vi "Lockin.Low Pass Filter.vi"(8 "error in (no error)":errorcluster, 11 "DSP in":refnum<class "DSP.lvclass">) -> (0 "error out":errorcluster, 3 "DSP out":refnum<class "DSP.lvclass">)   [LabVIEW 2019, in "DSP.lvclass"]
uses:
  DSP.lvclass
  DSP.lvclass/DSP.ctl
panel:
  out "Waveforms out":T1
  out "Waveforms in":T1
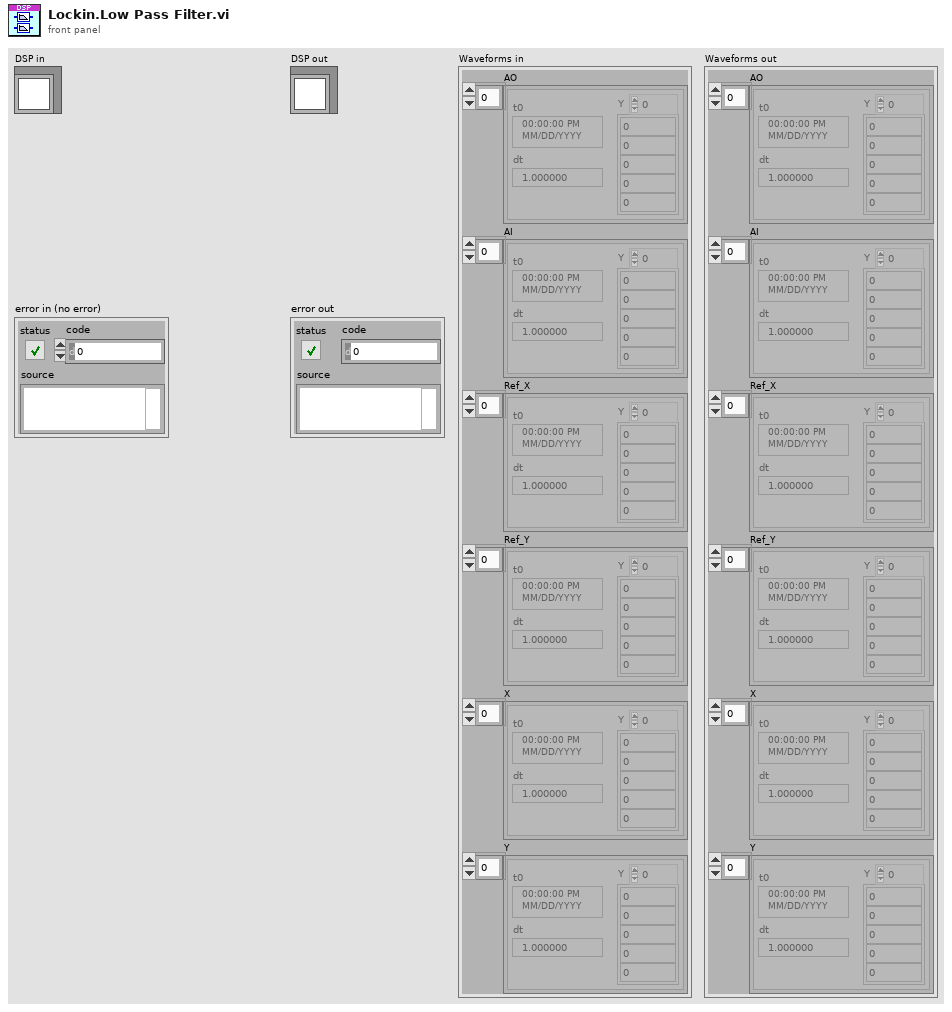
[diagram p1: front panel]
types:
  T1 = cluster{"AO":waveform(dbl)[], "AI":waveform(dbl)[], "Ref_X":waveform(dbl)[], "Ref_Y":waveform(dbl)[], "X":waveform(dbl)[], "Y":waveform(dbl)[]}
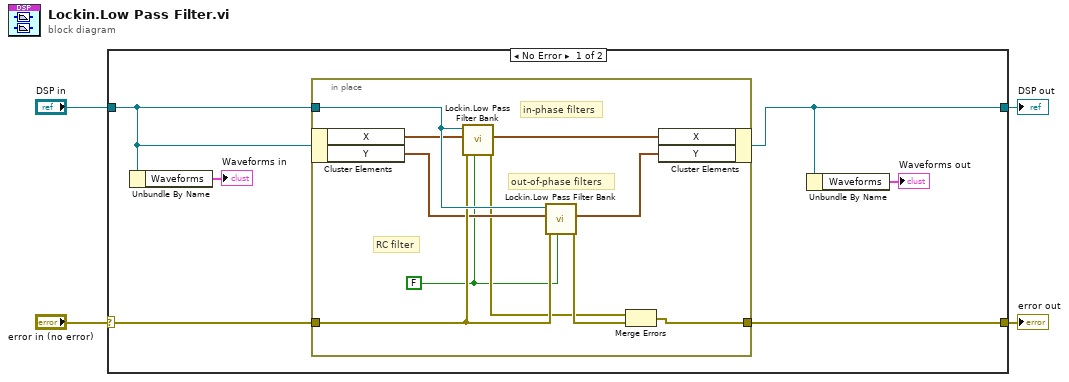
[diagram p0: block diagram]
diagram:
  n1 = case shown="No Error" "error in (no error)" {
    selector: "error in (no error)" -> [w9 w22]
    tunnel: [w10 w22] -> w4
    tunnel: [w5 w21] -> w3
    tunnel: "DSP in" -> [w7 w21]
    frame No Error {
      n2 = Unbundle By Name(w7) -> ("Waveforms"=→"Waveforms in":T1)
      n3 = in-place {
        in-place-border: [w20] -> w10
        in-place-border: w7 -> [w19]
        in-place-border: w9 -> [w18]
        w11 = FALSE ("Butterworth? [T]")
        # "RC filter"
        # "out-of-phase filters"
        # "in-phase filters"
        n4 = in-place-cluster #1(w7) -> ("X"=w17:waveform(dbl)[], "Y"=w16:waveform(dbl)[])
        n5 = call "Lockin.Low Pass Filter Bank.vi"("Butterworth? [T]"=w11, "error in (no error)"=w18, "WFms in"=w17, "DSP in"=w19) -> ("error out"=w14:errorcluster, "Wfms out"=w12:waveform(dbl)[])  [unwired: 6 in]
        n6 = call "Lockin.Low Pass Filter Bank.vi"("Butterworth? [T]"=w11, "error in (no error)"=w18, "WFms in"=w16, "DSP in"=w19) -> ("error out"=w15:errorcluster, "Wfms out"=w13:waveform(dbl)[])  [unwired: 6 in]
        n7 = Merge Errors(w14, w15) -> (w20:errorcluster)
        n8 = in-place-cluster #1("X"=w12, "Y"=w13) -> (w5:refnum<class "DSP.lvclass">)
      }
      n9 = Unbundle By Name(w5) -> ("Waveforms"=→"Waveforms out":T1)
    }
    frame Error {
    }
  }
  "error out" <- w4
  "DSP out" <- w3
